vi "Test Bench.vi"() -> ()   [LabVIEW 2018, in "TwinCAT ADS.lvclass"]
uses:
  TwinCAT ADS.lvclass
  TwinCAT.Ads
panel:
  out "Out Params":variant[](array[variant])
  out "Return":variant
  out "x-y":dbl format="%^#_6e"
  out "*(type *) &x":u8[](array[numeric])
  out "Byte Stream":u8[](array[numeric])
  # "21.7E-6"
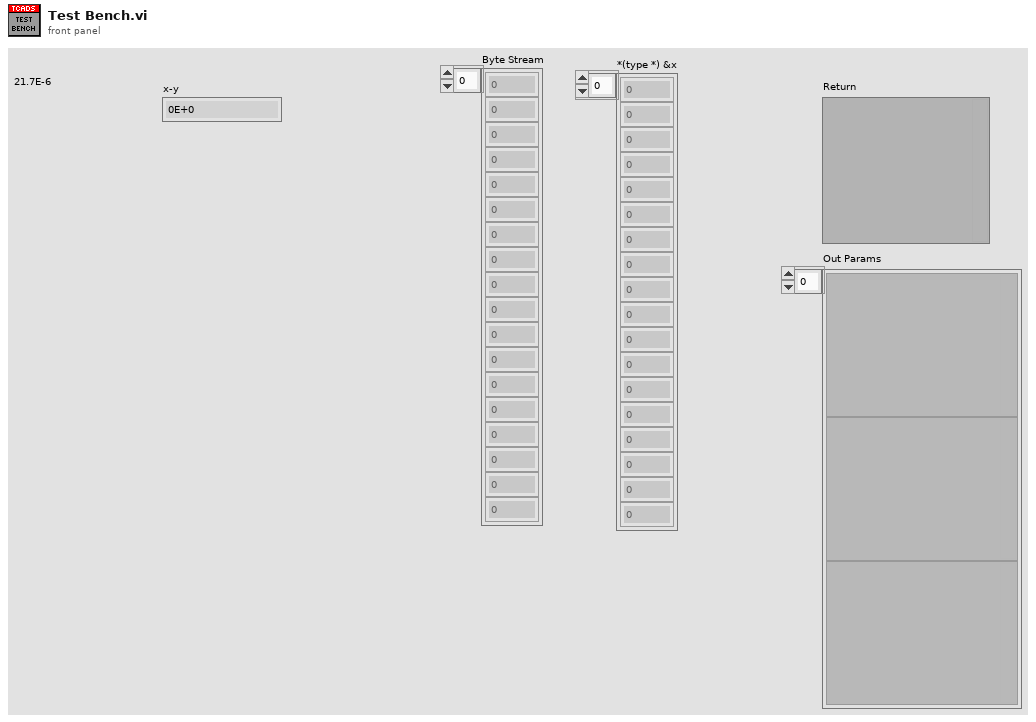
[diagram p1: front panel]
types:
  T1 = enum16{"big-endian, network order", "native, host order", "little-endian"}
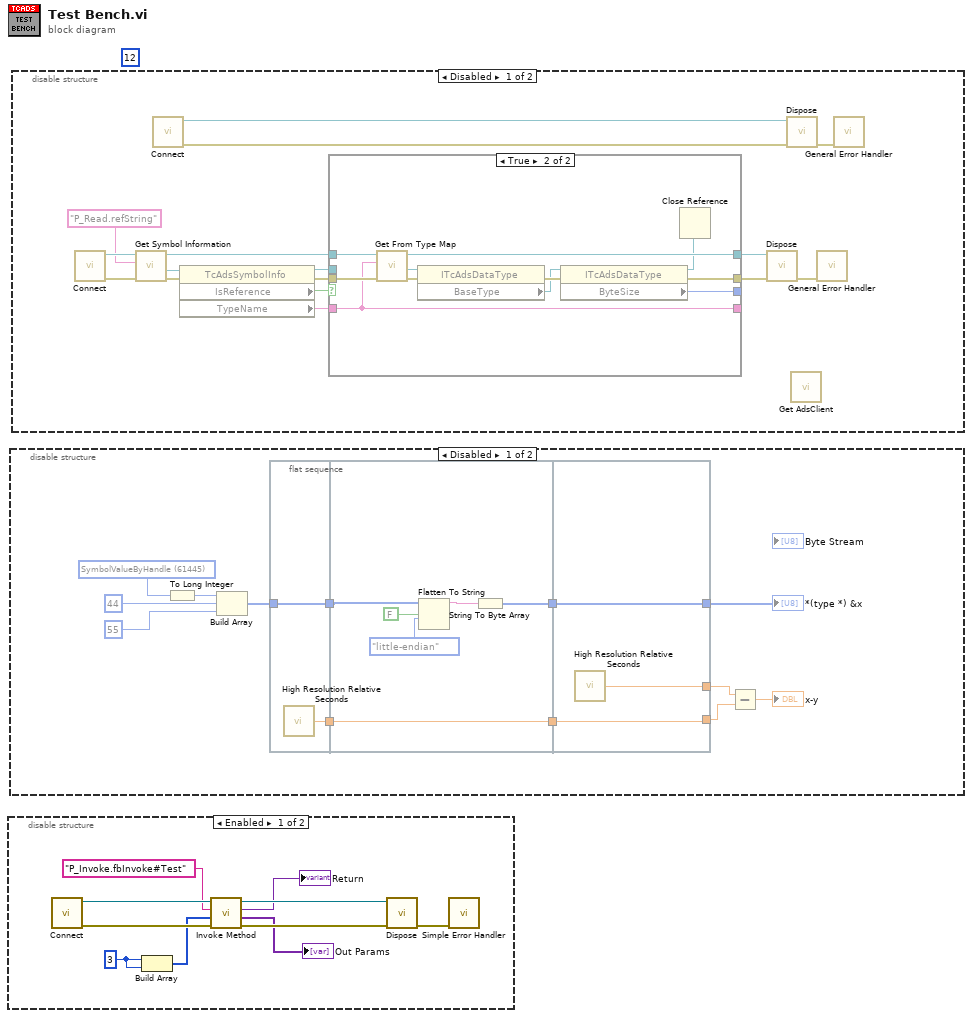
[diagram p0: block diagram]
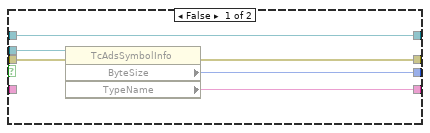
[diagram p4: hidden frame]
diagram:
  (unwired) i16 12
  n1 = disable-structure shown="Enabled" {
    frame Enabled {
      w1 = 3
      n2 = call "Connect.vi"() -> ("error out"=w8:errorcluster, "TwinCAT ADS out"=w9:refnum<class "TwinCAT ADS.lvclass">)  [unwired: 10 in]
      n3 = Build Array(w1, w1) -> (w2:i32[])
      n4 = call "Invoke Method.vi"("error in (no error)"=w8, "In Parameters"=w2, "Function Block#Method"="P_Invoke.fbInvoke#Test", "TwinCAT ADS in"=w9) -> ("error out"=w7:errorcluster, "Out Parameters"=→"Out Params":variant[], "Return"=→"Return":variant, "TwinCAT ADS out"=w6:refnum<class "TwinCAT ADS.lvclass">)  [unwired: 4 in]
      n5 = call "Dispose.vi"("error in (no error)"=w7, "TwinCAT ADS in"=w6) -> ("error out"=w10:errorcluster)  [unwired: 9 in]
      n6 = call <vilib>:"Simple Error Handler.vi"("error in (no error)"=w10) -> ()  [unwired: 4 in, 5 out]
    }
    frame Disabled {
    }
  }
  n7 = disable-structure shown="Disabled" {
    frame Disabled {
      w16 = u32 61445 items=["PlcRWIB"=16384, "PlcRWOB"=16400, "PlcRWMB"=16416, "PlcRWRB"=16432, "PlcRWDB"=16448, "SymbolTable"=61440, "SymbolName"=61441, "SymbolValue"=61442, "SymbolHandleByName"=61443, "SymbolValueByName"=61444, "SymbolValueByHandle"=61445, "SymbolReleaseHandle"=61446, "SymbolInfoByName"=61447, "SymbolVersion"=61448, "SymbolInfoByNameEx"=61449, "SymbolDownload"=61450, "SymbolUpload"=61451, "SymbolUploadInfo"=61452, "SymbolNote"=61456, "IOImageRWIB"=61472, "IOImageRWIX"=61473, "IOImageRWOB"=61488, "IOImageRWOX"=61489, "IOImageClearI"=61504, "IOImageClearO"=61520, "SumCommandRead"=61568, "SumCommandWrite"=61569, "SumCommandReadWrite"=61570, "SumCommandReadEx"=61571, "SumCommandReadEx2"=61572, "SumCommandAddDevNote"=61573, "SumCommandDelDevNote"=61574, "DeviceData"=61696] ("SumCommandRead")
      n8 = To Long Integer(number=w16) -> (32bit integer=w17:i32)
      n9 = Build Array(w17, 44 ("Handle"), 55 ("ByteSize")) -> (w15:i32[])
      n10 = flat-sequence {
        tunnel: w15 -> [w25]
        tunnel: [w25] -> w23
        tunnel: [w24] -> w22
        tunnel: w23 -> [w28]
        tunnel: [w26] -> w21
        tunnel: w22 -> [w31]
        tunnel: [w31] -> w20
        tunnel: [w34] -> w11
        tunnel: w21 -> [w34]
        tunnel: w20 -> [w33]
        tunnel: [w33] -> w13
        tunnel: [w32] -> w14
        frame #0 {
          n11 = call <vilib>:"High Resolution Relative Seconds.vi"() -> ("relative seconds"=w24:dbl)
        }
        frame #1 {
          n12 = Flatten To String(anything=w28, prepend array or string size? (T)=FALSE, byte order (0:big-endian, network order)=T1."little-endian" ("Byte Order (little-endian)")) -> (data string=w27:string)  [unwired: 1 in, 2 out]
          n13 = String To Byte Array(string=w27) -> (unsigned byte array=w26:u8[])
        }
        frame #2 {
          n14 = call <vilib>:"High Resolution Relative Seconds.vi"() -> ("relative seconds"=w32:dbl)
        }
      }
      n15 = Subtract(x=w14, y=w13) -> (x-y=→"x-y":dbl)
      "*(type *) &x" <- w11
    }
    frame Enabled {
    }
  }
  n16 = disable-structure shown="Disabled" {
    frame Disabled {
      n17 = call "Connect.vi"() -> ("error out"=w46:errorcluster, "TwinCAT ADS out"=w47:refnum<class "TwinCAT ADS.lvclass">)  [unwired: 10 in]
      n18 = call "Get Symbol Information.vi"("error in (no error)"=w46, "Symbol Name"="P_Read.refString", "TwinCAT ADS in"=w47) -> ("error out"=w49:errorcluster, ".NET Symbol Information"=w48:refnum<k24>, "TwinCAT ADS out"=w43:refnum<class "TwinCAT ADS.lvclass">)  [unwired: 6 in]
      n19 = call "Connect.vi"() -> ("error out"=w36:errorcluster, "TwinCAT ADS out"=w37:refnum<class "TwinCAT ADS.lvclass">)  [unwired: 10 in]
      n20 = property class="TcAdsSymbolInfo"(reference=w48, error in=w49) -> (reference out=w38:refnum<k24>, error out=w42:errorcluster, "IsReference"=w44:bool, "TypeName"=w40:string)
      n21 = case shown="True" w44 {
        tunnel: w43 -> [w56 w67]
        tunnel: w42 -> [w55 w66]
        tunnel: [w56 w62] -> w41
        tunnel: w40 -> [_ w63]
        tunnel: [w51 w63] -> _
        tunnel: [w52 w59] -> _
        tunnel: [w53 w57] -> w39
        tunnel: w38 -> [w54 _]
        frame False {
          n22 = property class="TcAdsSymbolInfo"(reference=w54, error in=w55) -> (error out=w53:errorcluster, "ByteSize"=w52:i32, "TypeName"=w51:string)  [unwired: 1 out]
        }
        frame True {
          n23 = call "Get From Type Map.vi"("error in (no error)"=w66, "Type Name"=w63, "TwinCAT ADS in"=w67) -> ("error out"=w65:errorcluster, ".NET AdsDataType"=w64:refnum<k24>, "TwinCAT ADS out"=w62:refnum<class "TwinCAT ADS.lvclass">)  [unwired: 6 in]
          n24 = property class="ITcAdsDataType"(reference=w64, error in=w65) -> (error out=w61:errorcluster, "BaseType"=w60:refnum<k24>)  [unwired: 1 out]
          n25 = property class="ITcAdsDataType"(reference=w60, error in=w61) -> (reference out=w58:refnum<k24>, error out=w57:errorcluster, "ByteSize"=w59:i32)
          n26 = Close Reference(reference=w58) -> ()  [unwired: 1 in, 1 out]
        }
      }
      n27 = call "Dispose.vi"("error in (no error)"=w39, "TwinCAT ADS in"=w41) -> ("error out"=w50:errorcluster)  [unwired: 9 in]
      n28 = call "Dispose.vi"("error in (no error)"=w36, "TwinCAT ADS in"=w37) -> ("error out"=w35:errorcluster)  [unwired: 9 in]
      n29 = call "Get AdsClient.vi"() -> ()  [unwired: 9 in, 3 out]
      n30 = call <vilib>:"General Error Handler.vi"("error in (no error)"=w50) -> ()  [unwired: 10 in, 5 out]
      n31 = call <vilib>:"General Error Handler.vi"("error in (no error)"=w35) -> ()  [unwired: 10 in, 5 out]
    }
    frame Enabled {
    }
  }
